vi "FuncVI-vhReset.vi"(5 "InstanceRef":T2, 9 "arg list":T1[](array[typedef]) {"num" format="%.2f"}) -> (0 "error out":bool, 3 "result":T1 {"num" format="%.2f"})   [LabVIEW 2021]
doc: "::: CalcExpress Toolkit :::\nCopyright (c) 2000-2026 Konstantin Shifershteyn. All rights reserved."
uses:
  cetypes.llb/CalcExpress Function Argument Info.ctl
  cetypes.llb/CalcExpress Instance RefNum.ctl
panel:
  in  "max arg num":i32=2
  in  "min arg num":i32=1
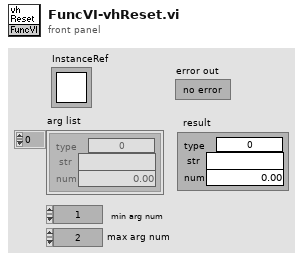
[diagram p1: front panel]
types:
  T1 = typedef "CalcExpress Function Argument Info.ctl" = cluster{"type":u32, "str":string, "num":dbl}
  T2 = typedef "CalcExpress Instance RefNum.ctl" = refnum<k1>
  T3 = enum32{"String", "DBL Number", "identifier", "1D Array of DBL", "2D Array of DBL", "CDB Number", "1D Array of CDB", "2D Array of CDB", "1D Array of String", "2D Array of String", "Unknown data type"}
  T4 = cluster{"index":i32, "data type":enum32{"String", "DBL Number", "identifier", "1D Array of DBL", "2D Array of DBL", "CDB Number", "1D Array of CDB", "2D Array of CDB", "1D Array of String", "2D Array of String", "Unknown data type"}, "default num":dbl, "default str":string}[]
  T5 = enum32{"nop", "create", "destroy", "reset", "get info", "config", "create_wrid"}
  T6 = typedef "VarMan Variable Context Handle.ctl" = i32
  T7 = cluster{"data type":enum32{"String", "DBL Number", "identifier", "1D Array of DBL", "2D Array of DBL", "CDB Number", "1D Array of CDB", "2D Array of CDB", "1D Array of String", "2D Array of String", "Unknown data type"}, string, dbl}
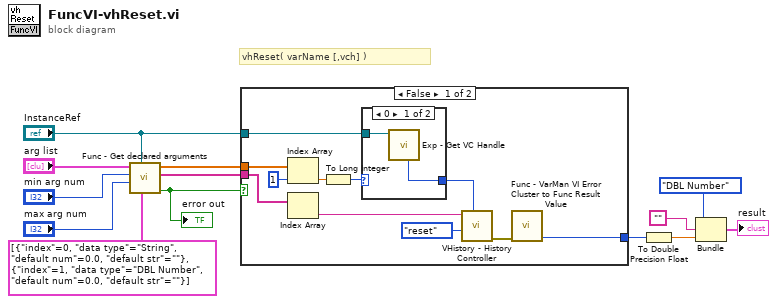
[diagram p0: block diagram]
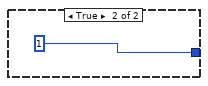
[diagram p3: hidden frame]
diagram:
  # "vhReset( varName [,vch] )"
  n1 = call "Func - Get declared arguments.vi"("arg descriptors"=T4 [{"index"=0, "data type"=enum."String", "default num"=0.0, "default str"=""}, {"index"=1, "data type"=enum."DBL Number", "default num"=0.0, "default str"=""}], "InstanceRef"="InstanceRef", "max arg num"="max arg num", "min arg num"="min arg num", "arg list"="arg list") -> ("error out"=w12:bool, "str list"=w8:string[], "num list"=w1:dbl[])  [unwired: 3 in, 1 out]
  "error out" <- w12
  n2 = case shown="False" w12 {
    tunnel: w1 -> [w21 _]
    tunnel: w8 -> [w24 _]
    tunnel: [w14 1 ("code")] -> w7
    tunnel: "InstanceRef" -> [w19 _]
    frame False {
      n3 = Index Array(array=w21, index=1) -> (element=w20:dbl)
      n4 = Index Array(array=w24) -> (element=w23:string)  [unwired: 1 in]
      n5 = To Long Integer(number=w20) -> (32bit integer=w18:i32)
      n6 = case shown="0" w18 {
        selector: w18 -> [_ w27]
        tunnel: w19 -> [w26 _]
        tunnel: [w25 w27] -> w17
        frame 0 {
          n7 = call "Exp - Get VC Handle.vi"("InstanceRef"=w26) -> ("VC Handle"=w25:T6)  [unwired: 5 in, 3 out]
        }
        frame Default {
        }
      }
      n8 = call "VHistory - History Controller.vi"("VC Handle"=w17, "cmd (nop:default)"=T5."reset", "name_spec"=w23) -> ("error out"=w15:errorcluster)  [unwired: 5 in, 3 out]
      n9 = call "Func - VarMan VI Error Cluster to Func Result Value.vi"("VarMan VI error in"=w15) -> ("CE Function Result Value"=w14:i32)  [unwired: 10 in]
    }
    frame True {
    }
  }
  n10 = To Double Precision Float(number=w7) -> (double precision float=w6:dbl)
  n11 = Bundle("data type"=T3."DBL Number", "", w6) -> (→"result":T7)  [unwired: 1 in]
